vi "RemoteVI Running Panels.vi"(0 "hWnds":u64[](array[numeric]), 11 "error in":errorcluster) -> (4 "running panels":u64[](array[numeric]), 15 "error out":errorcluster)   [LabVIEW 2020, in "RemoteVI.lvlib"]
doc: "Which of hWnds are front panel windows of VIs that are running - an application's own windows (a subVI panel opened with FP.Open or Show front panel when called, a second non-modal window) as opposed to IDE windows (Project Explorer, block diagrams, panels of VIs being edited), which Win32 cannot tell apart (all are LVDChild windows owned by LabVIEW's hidden frame window, measured on LabVIEW 2025). For every VI in memory of this application instance (Application:All VIs In Memory) whose Execution:State is running (Run Top Level or Running) and whose front panel is open, Front Panel Window:OS Window is compared with hWnds. A VI Server call: RemoteVI Track Windows.vi calls it only for windows that just appeared and only while no modal window is listed (about 60 ms for 400 VIs in memory, measured). The names are wired to Open VI Reference as strings; converted to paths, library members answered error 7 and the others error 1445 (measured). Errors of single VIs are skipped."
uses:
  RemoteVI.lvlib
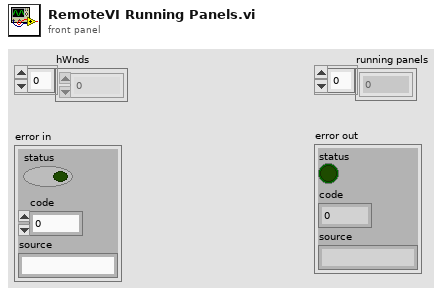
[diagram p1: front panel]
types:
  T1 = enum32{"Bad", "Idle", "Run top level", "Running"}
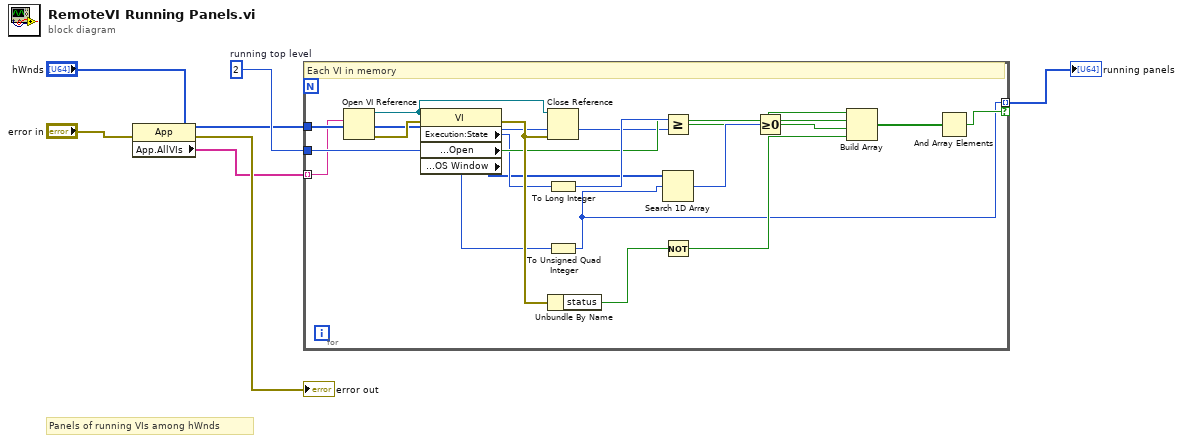
[diagram p0: block diagram]
diagram:
  w5 = 2  # running top level
  # "Panels of running VIs among hWnds"
  n1 = property class="App"(error in="error in") -> (error out=→"error out":errorcluster, "App.AllVIs"=w3:string[])  [unwired: 1 in, 1 out]
  n2 = for {
    tunnel: "hWnds" -> [w8]
    tunnel: w5 -> [w9]
    tunnel: w3 -> [w7] mode=indexing
    tunnel: [w18] -> w6 mode=indexing if=w24
    # "Each VI in memory"
    n3 = Open VI Reference(vi path=w7) -> (vi reference=w10:refnum<vi>, error out=w11:errorcluster)  [unwired: 5 in]
    n4 = property class="VI"(reference=w10, error in=w11) -> (error out=w15:errorcluster, "Execution:State"=w12:T1, "Front Panel Window:Open"=w13:bool, "Front Panel Window:OS Window"=w14:i32)  [unwired: 1 out]
    n5 = Close Reference(reference=w10, error in (no error)=w15) -> ()  [unwired: 1 out]
    n6 = To Long Integer(number=w12) -> (32bit integer=w16:i32)
    n7 = To Unsigned Quad Integer(1:w14) -> (0:w18:u64)
    n8 = Unbundle By Name(w15) -> ("status"=w21:bool)
    n9 = Greater Or Equal?(x=w16, y=w9) -> (x >= y?=w17:bool)
    n10 = Search 1D Array(1D array=w8, element=w18) -> (index of element=w19:i32)  [unwired: 1 in]
    n11 = Not(x=w21) -> (.not. x?=w22:bool)
    n12 = Greater Or Equal To 0?(x=w19) -> (x >= 0?=w20:bool)
    n13 = Build Array(w17, w13, w20, w22) -> (w23:bool[])
    n14 = And Array Elements(Boolean array=w23) -> (logical AND=w24:bool)
  }
  "running panels" <- w6
